vi "from string.vi"(8 "error in":errorcluster, 9 "data":string, 10 "version":string, 11 "SystemLin Tag Module configuration in":refnum<class "SystemLink configuration.lvclass">) -> (0 "error out":errorcluster, 3 "SystemLin Tag Module configuration out":refnum<class "SystemLink configuration.lvclass">)   [LabVIEW 2015, in "SystemLink configuration.lvclass"]
doc: "Provides an interface for loading a module configuration from a file or other serialized data source. It is recommended that all children of this class store data in two sets--data required for its own initialization, and any data required for parent initialization--and that each implementation uses the <b>Call Parent Method</b> primitive to de-serialize parent information. As a result, it is expected that every module configuration class calls <b>component configuration.lvclass:From String.vi</b>."
uses:
  SystemLink configuration.lvclass
  Connection Type.ctl
  <vilib>/NI/Tag Bus Module Framework/channel/TBM channel.lvclass
  Line.ctl
  Data Tag Type.ctl
  <vilib>/NI/Tag Bus/tag/tag descriptor.lvclass/tag descriptor.ctl
  SystemLink configuration.lvclass/SystemLink configuration.ctl
  Connection Configuration.ctl
  <vilib>/NI/Tag Bus Module Framework/module configuration/TBM module configuration.lvclass
  <vilib>/NI/Configuration Framework/serializable configuration/NISE_CEF_serializable configuration.lvclass
  <vilib>/NI/Tag Bus/tag/tag descriptor.lvclass
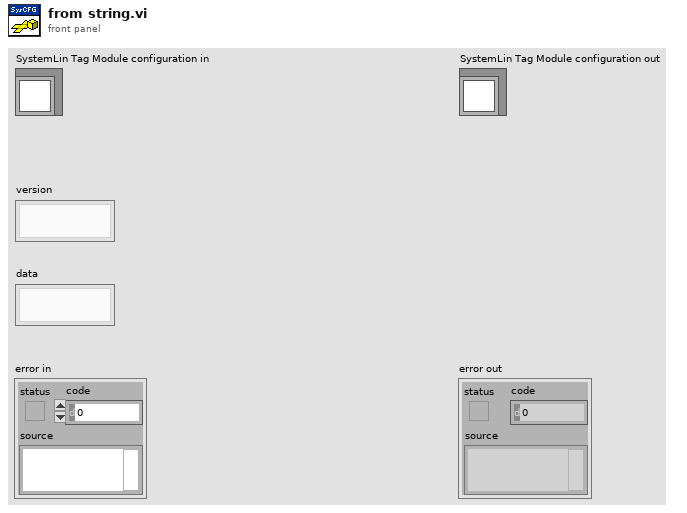
[diagram p1: front panel]
types:
  T1 = typedef "SystemLink configuration.lvclass/Connection Type.ctl" = enum16{"AMQP", "HTTP", "API Key (SystemLink Cloud)"}
  T2 = typedef "SystemLink configuration.lvclass/Line.ctl" = cluster{"channel":refnum<class "TBM channel.lvclass">, "Data Tag Type":T3}
  T3 = typedef "SystemLink configuration.lvclass/Data Tag Type.ctl" = enum16{"Double", "Single", "I32", "I16", "I8", "U64", "U32", "U16", "U8", "Boolean", "String", "Timestamp"}
  T4 = typedef "SystemLink configuration.lvclass/Connection Configuration.ctl" = cluster{"Connection Type":T1, "AMQP":cluster{"Configuration ID":string}, "HTTP":cluster{"Verify Server?":bool, "Server URL":string, "CA Certificate File":string, "User Info":cluster{"Username":string, "Password":string}, "API Key":string}}
  T5 = typedef "tag bus.lvlib/tag descriptor.lvclass/Data Type.ctl" = enum16{"Double", "Single", "I64", "I32", "I16", "I8", "U64", "U32", "U16", "U8", "Boolean", "String", "Array of Double", "Array of Single", "Array of I64", "Array of I32", "Array of I16", "Array of I8", "Array of U64", "Array of U32", "Array of U16", "Array of U8", "Array of Boolean", "Array of String"}
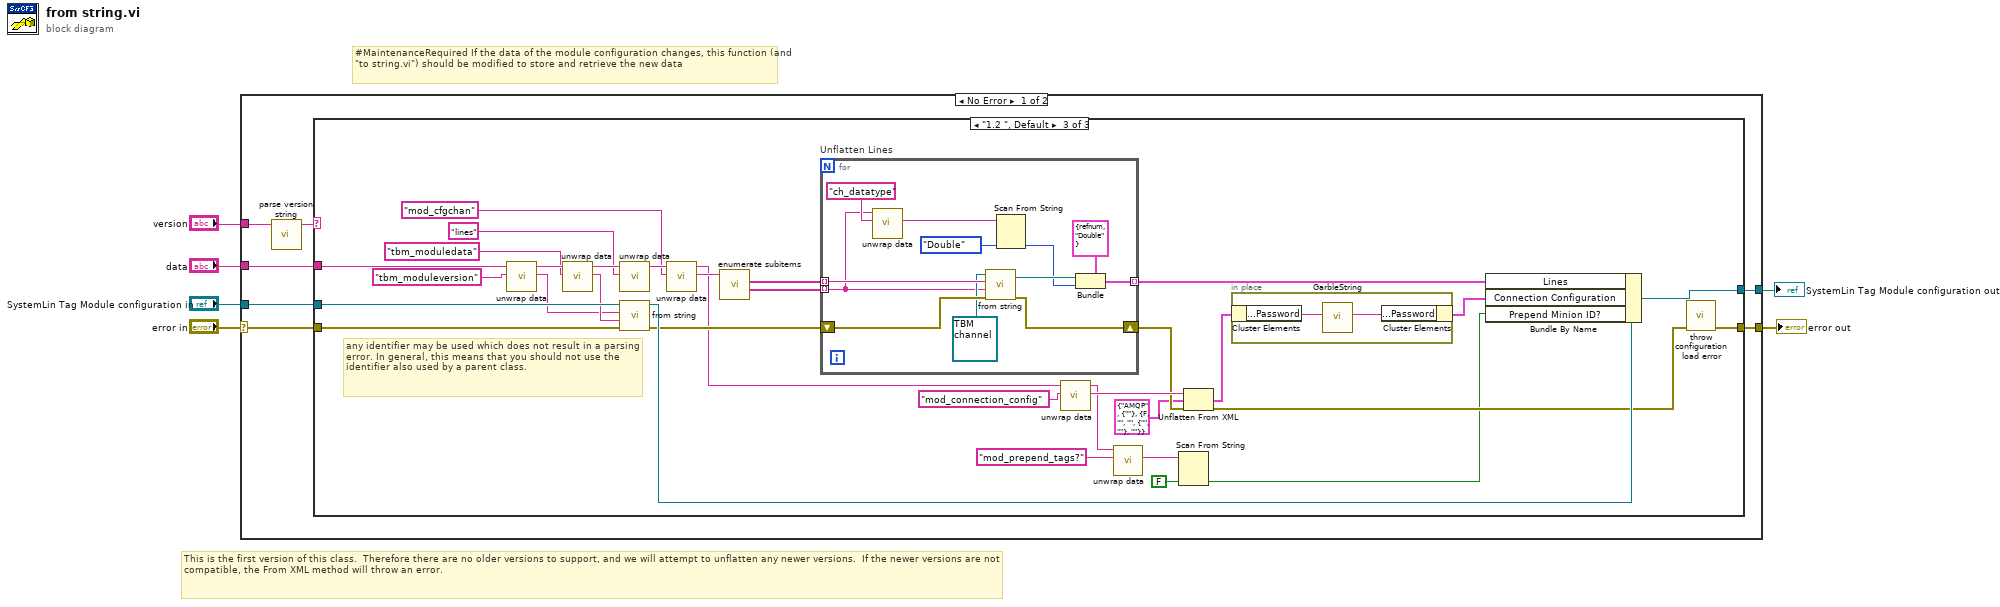
[diagram p0: block diagram]
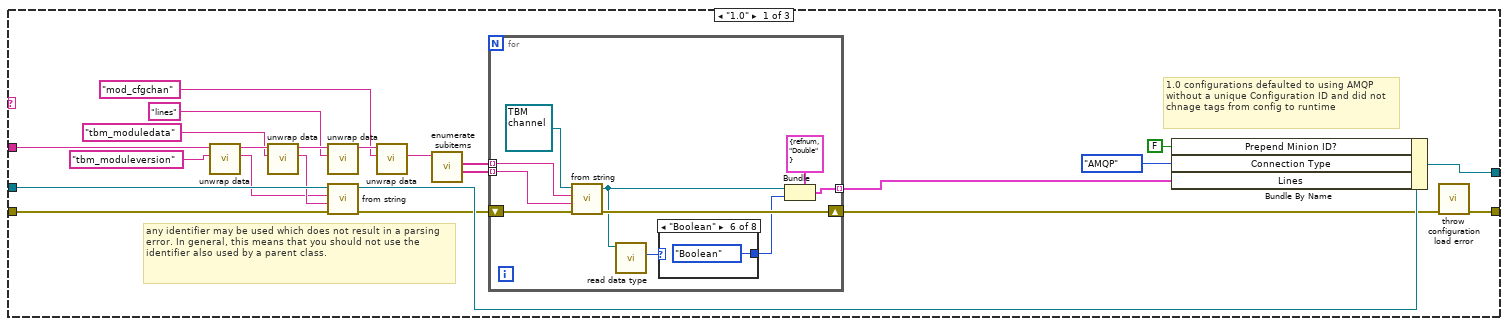
[diagram p2: hidden frame]
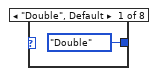
[diagram p3: hidden frame]
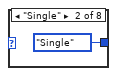
[diagram p4: hidden frame]
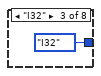
[diagram p5: hidden frame]
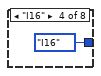
[diagram p6: hidden frame]
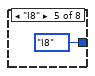
[diagram p7: hidden frame]
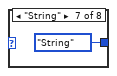
[diagram p8: hidden frame]
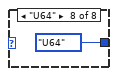
[diagram p9: hidden frame]
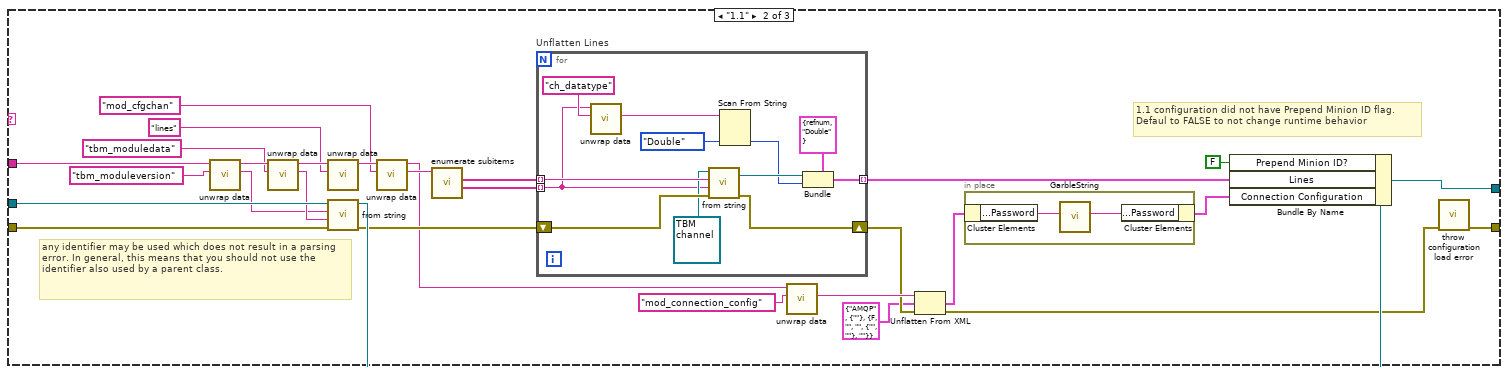
[diagram p10: hidden frame]
diagram:
  # "#MaintenanceRequired If the data of the module configuration changes, this function (and \"to string.vi\") should be modified to store and retrieve the new data"
  # "This is the first version of this class.  Therefore there are no older versions to support, and we will attempt to unflatten any newer versions.  If the newer versions are not compatible, the From XML method will throw an error."
  n1 = case shown="No Error" "error in" {
    selector: "error in" -> [w7 w146]
    tunnel: "data" -> [w13 _]
    tunnel: "SystemLin Tag Module configuration in" -> [w12 w145]
    tunnel: [w11 w145] -> w5
    tunnel: [w10 w146] -> w4
    tunnel: "version" -> [w9 _]
    frame No Error {
      n2 = call <vilib>:"parse version string.vi"("full version"=w9) -> ("major.minor version"=w8:string)  [unwired: 7 in, 3 out]
      n3 = case shown="\"1.2 \", Default" w8 {
        tunnel: w13 -> [w33 w80 w127]
        tunnel: w7 -> [w32 w79 w126]
        tunnel: w12 -> [w36 w83 w130]
        tunnel: [w24 w71 w118] -> w11
        tunnel: [w35 w82 w129] -> w10
        frame "1.0" {
          # "1.0 configurations defaulted to using AMQP without a unique Configuration ID and did not chnage tags from config to runtime"
          # "any identifier may be used which does not result in a parsing error. In general, this means that you should not use the identifier also used by a parent class."
          n4 = call <vilib>:"unwrap data.vi"("identifier"="tbm_moduleversion" ("additional identifier"), "data to unwrap"=w33) -> ("unwrapped data"=w28:string, "remaining string"=w34:string)  [unwired: 8 in]
          n5 = call <vilib>:"unwrap data.vi"("identifier"="tbm_moduledata" ("additional identifier"), "data to unwrap"=w34) -> ("unwrapped data"=w30:string, "remaining string"=w27:string)  [unwired: 8 in]
          n6 = call <vilib>:"unwrap data.vi"("identifier"="lines" ("additional identifier"), "data to unwrap"=w27) -> ("remaining string"=w23:string)  [unwired: 8 in, 1 out]
          n7 = call-parent "from string.vi"("error in"=w32, "data"=w30, "version"=w28, "module configuration in"=w36) -> ("error out"=w19:errorcluster, "module configuration out"=w25:refnum<class "SystemLink configuration.lvclass">)  [unwired: 6 in]
          n8 = call <vilib>:"unwrap data.vi"("identifier"="mod_cfgchan", "data to unwrap"=w23) -> ("unwrapped data"=w18:string)  [unwired: 8 in, 1 out]
          n9 = call <vilib>:"enumerate subitems.vi"("data to enumerate"=w18) -> ("associated data"=w20:string[], "discovered subitems"=w21:string[])  [unwired: 8 in, 1 out]
          n10 = for {
            shift-right: [w46] -> w16
            shift-left: w19 -> [w45]
            tunnel: w21 -> [w44] mode=indexing
            tunnel: w20 -> [w43] mode=indexing
            tunnel: [w40] -> w17 mode=indexing
            n11 = call-dynamic "from string.vi"("error in"=w45, "channel data"=w43, "identifier"=w44, "channel in"=refnum<class "TBM channel.lvclass"> refnum) -> ("error out"=w46:errorcluster, "channel out"=w39:refnum<class "TBM channel.lvclass">)  [unwired: 6 in]
            n12 = call <vilib>:"read data type.vi"("system tag in"=w39) -> ("data type"=w38:T5)  [unwired: 8 in, 2 out]
            n13 = case shown="\"Boolean\"" w38 {
              tunnel: [Data_Tag_Type."Double" ("Data Tag Type") Data_Tag_Type."Single" ("Data Tag Type") Data_Tag_Type."I32" ("Data Tag Type") Data_Tag_Type."I16" ("Data Tag Type") Data_Tag_Type."I8" ("Data Tag Type") Data_Tag_Type."Boolean" ("Data Tag Type") Data_Tag_Type."String" ("Data Tag Type") Data_Tag_Type."U64" ("Data Tag Type")] -> w37
              frame "Double", Default {
              }
              frame "Single" {
              }
              frame "I32" {
              }
              frame "I16" {
              }
              frame "I8" {
              }
              frame "Boolean" {
              }
              frame "String" {
              }
              frame "U64" {
              }
            }
            n14 = Bundle(cluster=T2 {"channel"=refnum, "Data Tag Type"=enum."Double"} ("Line"), "channel"=w39, "Data Tag Type"=w37) -> (w40:T2)
          }
          n15 = Bundle By Name(cluster=w25, "Prepend Minion ID?"=FALSE, "Connection Type"=Connection_Type."AMQP" ("Connection Configuration.Connection Type"), "Lines"=w17) -> (w24:refnum<class "SystemLink configuration.lvclass">)
          n16 = call <vilib>:"throw configuration load error.vi"("error in"=w16) -> ("error out"=w35:errorcluster)  [unwired: 10 in]
        }
        frame "1.1" {
          # "1.1 configuration did not have Prepend Minion ID flag. Defaul to FALSE to not change runtime behavior"
          # "any identifier may be used which does not result in a parsing error. In general, this means that you should not use the identifier also used by a parent class."
          n17 = call <vilib>:"unwrap data.vi"("identifier"="tbm_moduleversion" ("additional identifier"), "data to unwrap"=w80) -> ("unwrapped data"=w75:string, "remaining string"=w81:string)  [unwired: 8 in]
          n18 = call <vilib>:"unwrap data.vi"("identifier"="tbm_moduledata" ("additional identifier"), "data to unwrap"=w81) -> ("unwrapped data"=w77:string, "remaining string"=w74:string)  [unwired: 8 in]
          n19 = call <vilib>:"unwrap data.vi"("identifier"="lines" ("additional identifier"), "data to unwrap"=w74) -> ("remaining string"=w70:string)  [unwired: 8 in, 1 out]
          n20 = call-parent "from string.vi"("error in"=w79, "data"=w77, "version"=w75, "module configuration in"=w83) -> ("error out"=w66:errorcluster, "module configuration out"=w72:refnum<class "SystemLink configuration.lvclass">)  [unwired: 6 in]
          n21 = call <vilib>:"unwrap data.vi"("identifier"="mod_cfgchan", "data to unwrap"=w70) -> ("unwrapped data"=w65:string, "remaining string"=w63:string)  [unwired: 8 in]
          n22 = call <vilib>:"enumerate subitems.vi"("data to enumerate"=w65) -> ("associated data"=w67:string[], "discovered subitems"=w68:string[])  [unwired: 8 in, 1 out]
          n23 = for "Unflatten Lines" {
            shift-right: [w97] -> w60
            shift-left: w66 -> [w96]
            tunnel: w68 -> [w95] mode=indexing
            tunnel: w67 -> [w87] mode=indexing
            tunnel: [w91] -> w64 mode=indexing
            n24 = call <vilib>:"unwrap data.vi"("identifier"="ch_datatype", "data to unwrap"=w87) -> ("unwrapped data"=w86:string)  [unwired: 8 in, 1 out]
            n25 = call-dynamic "from string.vi"("error in"=w96, "channel data"=w87, "identifier"=w95, "channel in"=refnum<class "TBM channel.lvclass"> refnum) -> ("error out"=w97:errorcluster, "channel out"=w92:refnum<class "TBM channel.lvclass">)  [unwired: 6 in]
            n26 = Scan From String(input string=w86, default 1=Data_Tag_Type."Double" ("Data Tag Type")) -> (output 1=w88:T3)  [unwired: 3 in, 3 out]
            n27 = Bundle(cluster=T2 {"channel"=refnum, "Data Tag Type"=enum."Double"} ("Line"), "channel"=w92, "Data Tag Type"=w88) -> (w91:T2)
          }
          n28 = call <vilib>:"unwrap data.vi"("identifier"="mod_connection_config", "data to unwrap"=w63) -> ("unwrapped data"=w61:string)  [unwired: 8 in, 1 out]
          n29 = Unflatten From XML(xml string=w61, type=T4 {"Connection Type"=enum."AMQP", "AMQP"={"Configuration ID"=""}, "HTTP"={"Verify Server?"=FALSE, "Server URL"="", "CA Certificate File"="", "User Info"={"Username"="", "Password"=""}, "API Key"=""}} ("anything"), error in (no error)=w60) -> (value=w56:T4, error out=w59:errorcluster)
          n30 = in-place {
            n31 = in-place-cluster #1(w56) -> ("HTTP.User Info.Password"=w85:string)
            n32 = call "GarbleString.vi"("String In"=w85) -> ("String Out"=w84:string)  [unwired: 10 in]
            n33 = in-place-cluster #1("HTTP.User Info.Password"=w84) -> (w57:T4)
          }
          n34 = Bundle By Name(cluster=w72, "Prepend Minion ID?"=FALSE, "Lines"=w64, "Connection Configuration"=w57) -> (w71:refnum<class "SystemLink configuration.lvclass">)
          n35 = call <vilib>:"throw configuration load error.vi"("error in"=w59) -> ("error out"=w82:errorcluster)  [unwired: 10 in]
        }
        frame "1.2 ", Default {
          # "any identifier may be used which does not result in a parsing error. In general, this means that you should not use the identifier also used by a parent class."
          n36 = call <vilib>:"unwrap data.vi"("identifier"="tbm_moduleversion" ("additional identifier"), "data to unwrap"=w127) -> ("unwrapped data"=w122:string, "remaining string"=w128:string)  [unwired: 8 in]
          n37 = call <vilib>:"unwrap data.vi"("identifier"="tbm_moduledata" ("additional identifier"), "data to unwrap"=w128) -> ("unwrapped data"=w124:string, "remaining string"=w121:string)  [unwired: 8 in]
          n38 = call <vilib>:"unwrap data.vi"("identifier"="lines" ("additional identifier"), "data to unwrap"=w121) -> ("remaining string"=w117:string)  [unwired: 8 in, 1 out]
          n39 = call-parent "from string.vi"("error in"=w126, "data"=w124, "version"=w122, "module configuration in"=w130) -> ("error out"=w113:errorcluster, "module configuration out"=w119:refnum<class "SystemLink configuration.lvclass">)  [unwired: 6 in]
          n40 = call <vilib>:"unwrap data.vi"("identifier"="mod_cfgchan", "data to unwrap"=w117) -> ("unwrapped data"=w112:string, "remaining string"=w110:string)  [unwired: 8 in]
          n41 = call <vilib>:"enumerate subitems.vi"("data to enumerate"=w112) -> ("associated data"=w114:string[], "discovered subitems"=w115:string[])  [unwired: 8 in, 1 out]
          n42 = for "Unflatten Lines" {
            shift-right: [w144] -> w107
            shift-left: w113 -> [w143]
            tunnel: w115 -> [w142] mode=indexing
            tunnel: w114 -> [w134] mode=indexing
            tunnel: [w138] -> w111 mode=indexing
            n43 = call <vilib>:"unwrap data.vi"("identifier"="ch_datatype", "data to unwrap"=w134) -> ("unwrapped data"=w133:string)  [unwired: 8 in, 1 out]
            n44 = call-dynamic "from string.vi"("error in"=w143, "channel data"=w134, "identifier"=w142, "channel in"=refnum<class "TBM channel.lvclass"> refnum) -> ("error out"=w144:errorcluster, "channel out"=w139:refnum<class "TBM channel.lvclass">)  [unwired: 6 in]
            n45 = Scan From String(input string=w133, default 1=Data_Tag_Type."Double" ("Data Tag Type")) -> (output 1=w135:T3)  [unwired: 3 in, 3 out]
            n46 = Bundle(cluster=T2 {"channel"=refnum, "Data Tag Type"=enum."Double"} ("Line"), "channel"=w139, "Data Tag Type"=w135) -> (w138:T2)
          }
          n47 = call <vilib>:"unwrap data.vi"("identifier"="mod_connection_config", "data to unwrap"=w110) -> ("unwrapped data"=w108:string, "remaining string"=w102:string)  [unwired: 8 in]
          n48 = call <vilib>:"unwrap data.vi"("identifier"="mod_prepend_tags?", "data to unwrap"=w102) -> ("unwrapped data"=w99:string)  [unwired: 8 in, 1 out]
          n49 = Scan From String(input string=w99, default 1=FALSE) -> (output 1=w98:bool)  [unwired: 3 in, 3 out]
          n50 = Unflatten From XML(xml string=w108, type=T4 {"Connection Type"=enum."AMQP", "AMQP"={"Configuration ID"=""}, "HTTP"={"Verify Server?"=FALSE, "Server URL"="", "CA Certificate File"="", "User Info"={"Username"="", "Password"=""}, "API Key"=""}} ("anything"), error in (no error)=w107) -> (value=w103:T4, error out=w106:errorcluster)
          n51 = in-place {
            n52 = in-place-cluster #2(w103) -> ("HTTP.User Info.Password"=w132:string)
            n53 = call "GarbleString.vi"("String In"=w132) -> ("String Out"=w131:string)  [unwired: 10 in]
            n54 = in-place-cluster #2("HTTP.User Info.Password"=w131) -> (w104:T4)
          }
          n55 = Bundle By Name(cluster=w119, "Lines"=w111, "Connection Configuration"=w104, "Prepend Minion ID?"=w98) -> (w118:refnum<class "SystemLink configuration.lvclass">)
          n56 = call <vilib>:"throw configuration load error.vi"("error in"=w106) -> ("error out"=w129:errorcluster)  [unwired: 10 in]
        }
      }
    }
    frame Error {
    }
  }
  "error out" <- w4
  "SystemLin Tag Module configuration out" <- w5
